vi "VIH HelpGen - HTML - Insert CSS References.vi"(5 "HTML Folder":path, 7 "CSS Folder":path, 8 "error in":errorcluster, 10 "CSS files":path[](array[path]), 11 "HTML in":string) -> (0 "error out":errorcluster, 3 "HTML out":string)   [LabVIEW 2014]
doc: "::: VI Helpeks :::\nCopyright (c) 2000-2026 Konstantin Shifershteyn. All rights reserved."
panel:
  # "VI Helpeks\nCopyright (c) 2012-2026 Konstantin Shifershteyn"
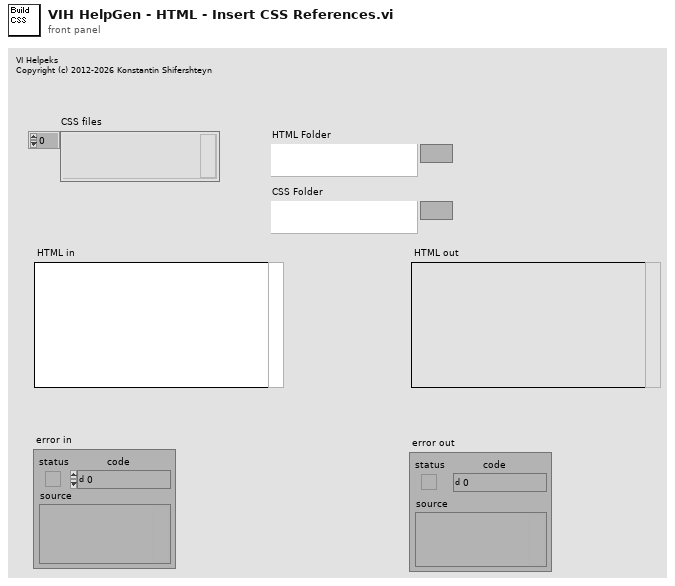
[diagram p1: front panel]
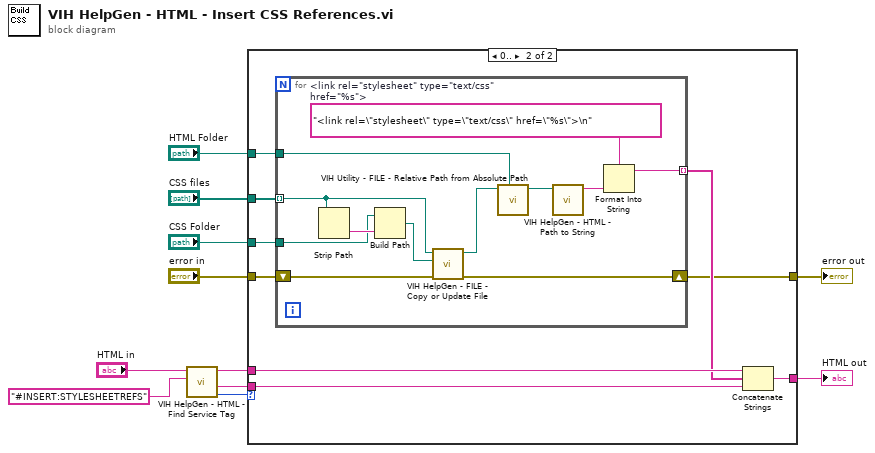
[diagram p0: block diagram]
diagram:
  n1 = call "VIH HelpGen - HTML - Find Service Tag.vi"("Tag name"="#INSERT:STYLESHEETREFS", "HTML in"="HTML in") -> ("Offset out"=w1:i32, "After"=w9:string, "Before"=w10:string)  [unwired: 6 in, 1 out]
  n2 = case shown="0.." w1 {
    tunnel: w10 -> [w12 w22]
    tunnel: w9 -> [_ w21]
    tunnel: [w12 w20] -> w8
    tunnel: "HTML Folder" -> [_ w18]
    tunnel: "CSS files" -> [_ w17]
    tunnel: "error in" -> [w13 w16]
    tunnel: "CSS Folder" -> [_ w15]
    tunnel: [w13 w14] -> w2
    frame ..-1 {
    }
    frame 0.. {
      n3 = for {
        tunnel: [w34] -> w19 mode=indexing
        tunnel: w18 -> [w33]
        tunnel: w17 -> [w27] mode=indexing
        shift-right: [w28] -> w14
        shift-left: w16 -> [w29]
        tunnel: w15 -> [w30]
        w32 = "<link rel=\"stylesheet\" type=\"text/css\" href=\"%s\">\n"  # <link rel="stylesheet" type="text/css" href="%s">
        n4 = Strip Path(path=w27) -> (name=w31:string)  [unwired: 1 out]
        n5 = Build Path(base path=w30, name or relative path=w31) -> (appended path=w26:path)
        n6 = call "VIH HelpGen - FILE - Copy or Update File.vi"("error in"=w29, "Target Path"=w26, "Source Path"=w27) -> ("error out"=w28:errorcluster, "Target Path out"=w25:path)  [unwired: 7 in]
        n7 = call "VIH Utility - FILE - Relative Path from Absolute Path.vi"("base path (empty: dir of Top VI)"=w33, "Path"=w25) -> ("Rel Path out"=w24:path)  [unwired: 7 in, 2 out]
        n8 = call "VIH HelpGen - HTML - Path to String.vi"("Path"=w24) -> ("String"=w23:string)  [unwired: 10 in]
        n9 = Format Into String(format string=w32, w23) -> (resulting string=w34:string)  [unwired: 2 in, 1 out]
      }
      n10 = Concatenate Strings(w22, w19, w21) -> (w20:string)
    }
  }
  "error out" <- w2
  "HTML out" <- w8
